vi "Shooter_Motor.vi"(0 "LeftMotorControlDevRef":T4={"DeviceStatus"={"status"=FALSE, "code"=0, "source"=""}, "Type"=enum."PWM", "PWM"={"PWM Channel"=enum."Invalid", "DeadBand"={"Name"="", "maxPositivePwm"=0, "minPositivePwm"=0, "centerPwm"=0, "maxNegativePwm"=0, "minNegativePwm"=0, "angularRange"=0}}, "CAN"={"Device Number"=0, "SetOutput VI Ref"=variant(refnum<vi> refnum), "GetOutput VI Ref"=variant(refnum<vi> refnum), "Enable VI Ref"=variant(refnum<vi> refnum), "Disable VI Ref"=variant(refnum<vi> refnum), "Data"=variant}, "Invert"=FALSE}, 1 "RightMotorControlDevRef":T4={"DeviceStatus"={"status"=FALSE, "code"=0, "source"=""}, "Type"=enum."PWM", "PWM"={"PWM Channel"=enum."Invalid", "DeadBand"={"Name"="", "maxPositivePwm"=0, "minPositivePwm"=0, "centerPwm"=0, "maxNegativePwm"=0, "minNegativePwm"=0, "angularRange"=0}}, "CAN"={"Device Number"=0, "SetOutput VI Ref"=variant(refnum<vi> refnum), "GetOutput VI Ref"=variant(refnum<vi> refnum), "Enable VI Ref"=variant(refnum<vi> refnum), "Disable VI Ref"=variant(refnum<vi> refnum), "Data"=variant}, "Invert"=FALSE}, 2 "ShooterSpeed":dbl format="%#_13g", 6 "Shooter_Forward?":bool) -> ()   [LabVIEW 2016]
uses:
  TypeDefs/ShooterPIDParameters_Type.ctl
  <vilib>/Rock Robotics/WPI/MotorControl/WPI_MotorControlDeviceRef.ctl
  <vilib>/Rock Robotics/WPI/MotorControl/WPI_MotorControlType.ctl
  <vilib>/Rock Robotics/SystemInterfaces/DIO/FPGA_DIOPWMChannel.ctl
  <vilib>/Rock Robotics/WPI/PWM/WPI_PWMDeadband.ctl
  TypeDefs/ShooterSpeed_Type.ctl
  <vilib>/Rock Robotics/WPI/ThirdParty/CanMotor/TalonSRX/WPI_CANTalonSRX_APIControlMode.ctl
  Global_Var-RefNum/Global_Var_Other.vi
panel:
  out "Waveform Chart 2":dbl(graph)
  out "Waveform Chart":T1(graph)
  in  "TargetVelocityPercent":dbl=0.9
  in  "PID Parameters":T2(tab)
  in  "3000rpm Params":T3={"F"=0.0, "P"=3.0, "I"=0.009, "D"=0.0, "IZone"=450.0, "RampRate"=0.0}
  in  "3500rpm Params":T3={"F"=0.0, "P"=3.0, "I"=0.008, "D"=0.0, "IZone"=350.0, "RampRate"=0.0}
  in  "4000rpm Params":T3={"F"=0.0, "P"=3.0, "I"=0.014, "D"=0.0, "IZone"=450.0, "RampRate"=0.0}
  in  "4500rpm Params":T3={"F"=0.0, "P"=3.0, "I"=0.013, "D"=0.0, "IZone"=450.0, "RampRate"=0.0}
  in  "5000rpm Params":T3={"F"=0.0, "P"=3.0, "I"=0.013, "D"=0.0, "IZone"=450.0, "RampRate"=0.0}
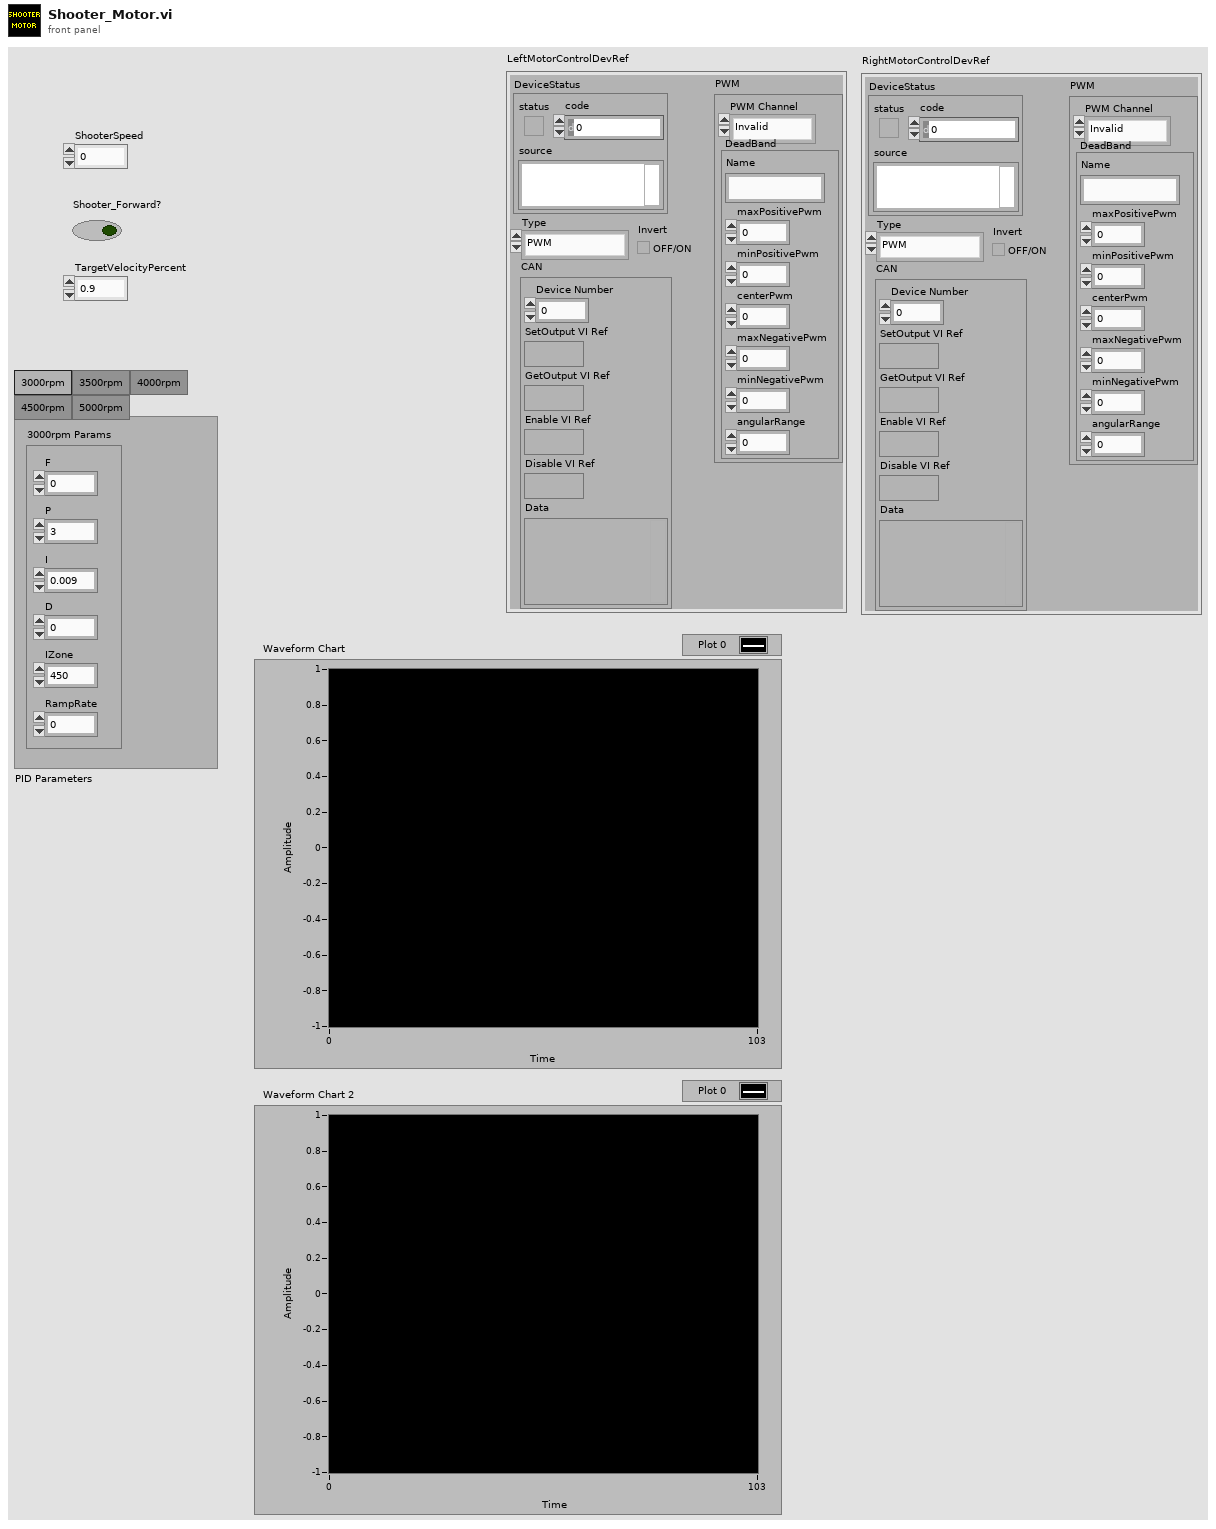
[diagram p1: front panel]
types:
  T1 = cluster{"ShooterSpeed":dbl, "Encoder Velocity":dbl, "Encoder Velocity":dbl}
  T2 = enum32{"3000rpm", "3500rpm", "4000rpm", "4500rpm", "5000rpm"}
  T3 = typedef "ShooterPIDParameters_Type.ctl" = cluster{"F":dbl, "P":dbl, "I":dbl, "D":dbl, "IZone":dbl, "RampRate":dbl}
  T4 = typedef "WPI_MotorControlDeviceRef.ctl" = cluster{"DeviceStatus":errorcluster, "Type":T5, "PWM":cluster{"PWM Channel":T6, "DeadBand":T7}, "CAN":cluster{"Device Number":u8, "SetOutput VI Ref":variant, "GetOutput VI Ref":variant, "Enable VI Ref":variant, "Disable VI Ref":variant, "Data":variant}, "Invert":bool}
  T5 = typedef "WPI_MotorControlType.ctl" = enum16{"PWM", "CAN"}
  T6 = typedef "FPGA_DIOPWMChannel.ctl" = enum8{"PWM 0", "PWM 1", "PWM 2", "PWM 3", "PWM 4", "PWM 5", "PWM 6", "PWM 7", "PWM 8", "PWM 9", "PWM MXP 0", "PWM MXP 1", "PWM MXP 2", "PWM MXP 3", "PWM MXP 4", "PWM MXP 5", "PWM MXP 6", "PWM MXP 7", "PWM MXP 8", "PWM MXP 9", "Invalid"}
  T7 = typedef "WPI_PWMDeadband.ctl" = cluster{"Name":string, "maxPositivePwm":i32, "minPositivePwm":i32, "centerPwm":i32, "maxNegativePwm":i32, "minNegativePwm":i32, "angularRange":u16}
  T8 = typedef "ShooterSpeed_Type.ctl" = enum16{"3000rpm", "3500rpm", "4000rpm", "4500rpm", "5000rpm", "FullPower"}
  T9 = typedef "WPI_CANTalonSRX_APIControlMode.ctl" = enum8{"Percent VBus", "Speed", "Position", "Slave", "Unchanged / Invalid", "Voltage Compensation", "Current", "Motion Profile", "Motion Magic"}
  T10 = typedef "WPI_CANTalonSRX_GlobalStatus.ctl" = cluster{"Applied Throttle":dbl, "Module Enabled":bool, "CAN Error":errorcluster, "Closed Loop Error":dbl, "Forward Limit Switch Closed":bool, "Reverse Limit Switch Closed":bool, "Sensor Position":dbl, "Sensor Velocity":dbl, "Current":dbl, "Sticky Fault - Over Temp":bool, "Sticky Fault - Under Voltage":bool, "Sticky Fault - Forward Limit":bool, "Sticky Fault - Reverse Limit":bool, "Sticky Fault - Forward Soft Limit":bool, "Sticky Fault - Reverse Soft Limit":bool, "Brake is Enabled":bool, "Encoder Position":dbl, "Encoder Velocity":dbl, "Encoder Index Count":dbl, "Encoder A Pin State":bool, "Encoder B Pin State":bool, "Encoder Index Pin State":bool, "Analog In":dbl, "Analog In Velocity":dbl, "Temperature (C)":dbl, "Battery Voltage":dbl, "Control 5 Is Supported":bool, "Current Profile Slot Select":dbl, "Pos Div 8":bool, "Vel Div 4":bool, "Pulse Width Position":i32, "Pulse Width Velocity":i32, "Pulse Width Rise To Rise (us)":i32, "Pulse Width Rise To Fall (us)":i32, "Mot Prof Active Is Under Run":bool, "Mot Prof Active Has Under Run":bool, "Mot Prof Active Is Last":bool, "Mot Prof Active Velocity Only":bool, "Mot Prof Active Is Valid":bool, "Mot Prof Buffer Is Full":bool, "Mot Prof Active Profile Slot Select":i32, "Mot Prof NextID":i32, "Mot Prof Count":i32, "Mot Prof Active Velocity":dbl, "Mot Prof Active Position":dbl, "Mot Prof Output Enable":i32}
  T11 = cluster{"ShooterSpeed":dbl, "Sensor Velocity":dbl, "Sensor Velocity":dbl}
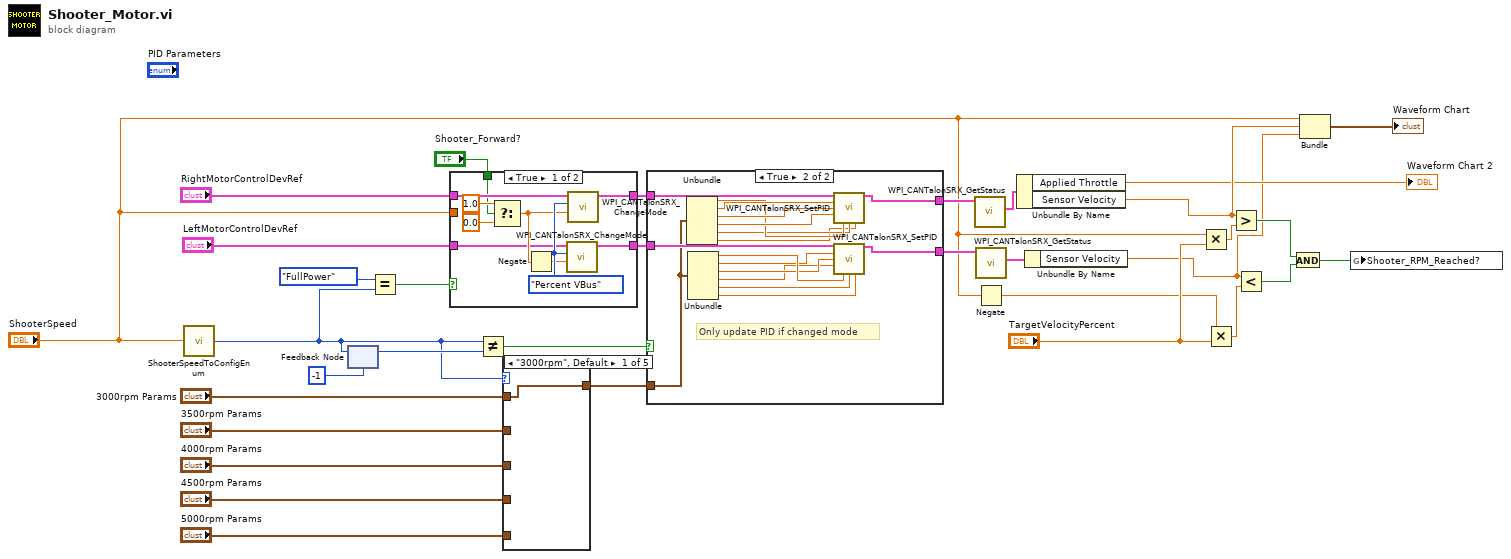
[diagram p0: block diagram]
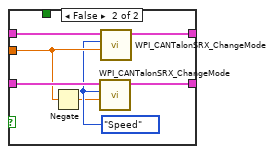
[diagram p2: hidden frame]
diagram:
  n1 = call "ShooterSpeedToConfigEnum.vi"("ShooterSpeed"="ShooterSpeed") -> ("ConfigEnum"=w3:T8)
  n2 = feedback-in #1(w3) -> ()
  n3 = feedback #1(-1) -> (w30:i32)
  n4 = Equal?(x=ShooterSpeed_Type."FullPower", y=w3) -> (x = y?=w1:bool)
  n5 = case shown="True" w1 {
    tunnel: "LeftMotorControlDevRef" -> [w38 w50]
    tunnel: "RightMotorControlDevRef" -> [w37 w49]
    tunnel: "ShooterSpeed" -> [_ w48]
    tunnel: [w36 w46] -> w23
    tunnel: [w35 w45] -> w22
    tunnel: "Shooter_Forward?" -> [w34 _]
    frame True {
      w43 = WPI_CANTalonSRX_APIControlMode."Percent VBus" ("Control Mode")
      n6 = Select(t=1.0, s=w34, f=0.0) -> (s? t:f=w40:dbl)
      n7 = Negate(x=w40) -> (-x=w39:dbl)
      n8 = call <vilib>:"WPI_CANTalonSRX_ChangeMode.vi"("Output"=w39, "Control Mode"=w43, "CAN Talon SRX Ref"=w38) -> ("CAN Talon SRX Ref"=w35:T4)  [unwired: 7 in, 1 out]
      n9 = call <vilib>:"WPI_CANTalonSRX_ChangeMode.vi"("Output"=w40, "Control Mode"=w43, "CAN Talon SRX Ref"=w37) -> ("CAN Talon SRX Ref"=w36:T4)  [unwired: 7 in, 1 out]
    }
    frame False {
      w47 = WPI_CANTalonSRX_APIControlMode."Speed" ("Control Mode")
      n10 = Negate(x=w48) -> (-x=w44:dbl)
      n11 = call <vilib>:"WPI_CANTalonSRX_ChangeMode.vi"("Output"=w44, "Control Mode"=w47, "CAN Talon SRX Ref"=w50) -> ("CAN Talon SRX Ref"=w45:T4)  [unwired: 7 in, 1 out]
      n12 = call <vilib>:"WPI_CANTalonSRX_ChangeMode.vi"("Output"=w48, "Control Mode"=w47, "CAN Talon SRX Ref"=w49) -> ("CAN Talon SRX Ref"=w46:T4)  [unwired: 7 in, 1 out]
    }
  }
  n13 = Not Equal?(x=w3, y=w30) -> (x != y?=w24:bool)
  n14 = case shown="\"3000rpm\", Default" w3 {
    tunnel: "3500rpm Params" -> [_ w52 _ _ _]
    tunnel: [w51 w52 w53 w54 w55] -> w11
    tunnel: "3000rpm Params" -> [w51 _ _ _ _]
    tunnel: "4000rpm Params" -> [_ _ w53 _ _]
    tunnel: "4500rpm Params" -> [_ _ _ w54 _]
    tunnel: "5000rpm Params" -> [_ _ _ _ w55]
    frame "3000rpm", Default {
    }
    frame "3500rpm" {
    }
    frame "4000rpm" {
    }
    frame "4500rpm" {
    }
    frame "5000rpm" {
    }
  }
  n15 = case shown="True" w24 {
    tunnel: w23 -> [w57 w74]
    tunnel: w22 -> [w56 w73]
    tunnel: w11 -> [_ w66]
    tunnel: [w57 w59] -> w14
    tunnel: [w56 w58] -> w13
    frame False {
    }
    frame True {
      # "Only update PID if changed mode"
      n16 = Unbundle(w66) -> ("F"=w69:dbl, "P"=w72:dbl, "I"=w71:dbl, "D"=w70:dbl, "IZone"=w68:dbl, "RampRate"=w67:dbl)
      n17 = Unbundle(w66) -> ("F"=w65:dbl, "P"=w64:dbl, "I"=w63:dbl, "D"=w62:dbl, "IZone"=w61:dbl, "RampRate"=w60:dbl)
      n18 = call <vilib>:"WPI_CANTalonSRX_SetPID.vi"("CAN Talon SRX Ref"=w74, "P"=w72, "I"=w71, "D"=w70, "F"=w69, "I Zone"=w68, "Ramp Rate"=w67) -> ("CAN Talon SRX Ref"=w59:T4)  [unwired: 7 in, 1 out]
      n19 = call <vilib>:"WPI_CANTalonSRX_SetPID.vi"("CAN Talon SRX Ref"=w73, "P"=w64, "I"=w63, "D"=w62, "F"=w65, "I Zone"=w61, "Ramp Rate"=w60) -> ("CAN Talon SRX Ref"=w58:T4)  [unwired: 7 in, 1 out]
    }
  }
  n20 = call <vilib>:"WPI_CANTalonSRX_GetStatus.vi"("CAN Talon SRX Ref"=w14) -> ("Talon SRX Status"=w21:T10)  [unwired: 8 in, 2 out]
  n21 = call <vilib>:"WPI_CANTalonSRX_GetStatus.vi"("CAN Talon SRX Ref"=w13) -> ("Talon SRX Status"=w17:T10)  [unwired: 8 in, 2 out]
  n22 = Negate(x="ShooterSpeed") -> (-x=w16:dbl)
  n23 = Unbundle By Name(w21) -> ("Applied Throttle"=→"Waveform Chart 2":dbl, "Sensor Velocity"=w27:dbl)
  n24 = Unbundle By Name(w17) -> ("Sensor Velocity"=w6:dbl)
  n25 = Multiply(x="ShooterSpeed", y="TargetVelocityPercent") -> (x*y=w20:dbl)
  n26 = Multiply(x=w16, y="TargetVelocityPercent") -> (x*y=w18:dbl)
  n27 = Greater?(x=w27, y=w20) -> (0:w19:bool)
  n28 = Less?(x=w6, y=w18) -> (x < y?=w15:bool)
  n29 = And(x=w19, y=w15) -> (x .and. y?=w29:bool)
  n30 = Bundle("ShooterSpeed"="ShooterSpeed", "Sensor Velocity"=w27, "Sensor Velocity"=w6) -> (→"Waveform Chart":T11)  [unwired: 1 in]
  n31 = global write "Global_Var_Other.vi" "Shooter_RPM_Reached?"(w29) -> ()
